vi "FuncVI-APSpectrum.vi"(5 "InstanceRef":T2, 9 "arg list":T1[](array[typedef]) {"num" format="%.2f"}) -> (0 "error out":bool, 3 "result":T1 {"num" format="%.2f"})   [LabVIEW 2021]
doc: "::: CalcExpress Toolkit :::\nCopyright (c) 2000-2026 Konstantin Shifershteyn. All rights reserved."
uses:
  cetypes.llb/CalcExpress Function Argument Info.ctl
  cetypes.llb/CalcExpress Instance RefNum.ctl
  <vilib>/Analysis/NI_AALPro.lvlib
panel:
  in  "max arg num":i32=3
  in  "min arg num":i32=2
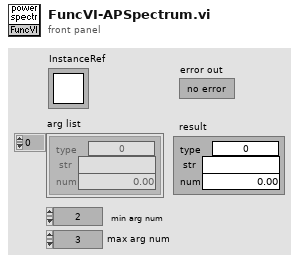
[diagram p1: front panel]
types:
  T1 = typedef "CalcExpress Function Argument Info.ctl" = cluster{"type":u32, "str":string, "num":dbl}
  T2 = typedef "CalcExpress Instance RefNum.ctl" = refnum<k1>
  T3 = enum8{"String", "DBL Number", "identifier", "1D Array of DBL", "2D Array of DBL", "CDB Number", "1D Array of CDB", "2D Array of CDB", "1D Array of String", "2D Array of String", "Unknown data type"}
  T4 = cluster{"index":i32, "type":enum8{"String", "DBL Number", "identifier", "1D Array of DBL", "2D Array of DBL", "CDB Number", "1D Array of CDB", "2D Array of CDB", "Unknown data type"}, "default num":dbl, "default str":string}[]
  T5 = typedef "VarMan Variable Context Handle.ctl" = i32
  T6 = cluster{"type":enum8{"String", "DBL Number", "identifier", "1D Array of DBL", "2D Array of DBL", "CDB Number", "1D Array of CDB", "2D Array of CDB", "1D Array of String", "2D Array of String", "Unknown data type"}, string, "df":dbl}
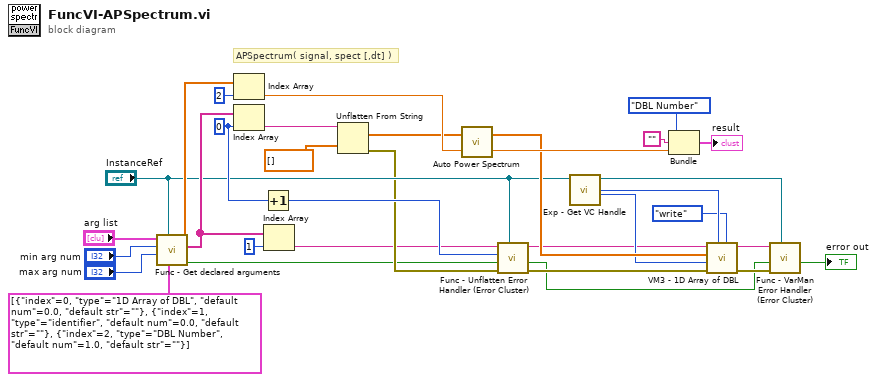
[diagram p0: block diagram]
diagram:
  w19 = 0
  # "APSpectrum( signal, spect [,dt] )"
  n1 = call "Func - Get declared arguments.vi"("arg descriptors"=T4 [{"index"=0, "type"=enum."1D Array of DBL", "default num"=0.0, "default str"=""}, {"index"=1, "type"=enum."identifier", "default num"=0.0, "default str"=""}, {"index"=2, "type"=enum."DBL Number", "default num"=1.0, "default str"=""}] ("args descriptors"), "InstanceRef"="InstanceRef", "max arg num"="max arg num", "min arg num"="min arg num", "arg list"="arg list") -> ("error out"=w5:bool, "str list"=w27:string[], "num list"=w25:dbl[])  [unwired: 3 in, 1 out]
  n2 = Index Array(array=w25, index=2) -> (element=w26:dbl)
  n3 = Index Array(array=w27, index=w19) -> (element=w22:string)
  n4 = Increment(x=w19) -> (x+1=w7:i32)
  n5 = Index Array(array=w27, index=1) -> (element=w4:string)
  n6 = Unflatten From String(type=dbl[] [] ("num list"), binary string=w22) -> (value=w20:dbl[], error out=w6:errorcluster)  [unwired: 3 in, 1 out]
  n7 = call <vilib>:"Auto Power Spectrum.vi"("dt"=w26, "Signal (V)"=w20) -> ("df"=w31:dbl, "Power Spectrum (V^2 rms)"=w14:dbl[])
  n8 = call "Func - Unflatten Error Handler (Error Cluster).vi"("InstanceRef"="InstanceRef", "Unflatten Error Cluster"=w6, "error status before"=w5, "argument number"=w7, "name"=w4) -> ("Error Cluster out"=w9:errorcluster, "error status out"=w1:bool, "dup name"=w3:string)  [unwired: 4 in]
  n9 = call "Exp - Get VC Handle.vi"("InstanceRef"="InstanceRef") -> ("writer ID"=w13:u32, "dup InstanceRef"=w10:T2, "VC Handle"=w16:T5)  [unwired: 5 in, 1 out]
  n10 = Bundle("type"=T3."DBL Number", "", "df"=w31) -> (→"result":T6)  [unwired: 1 in]
  n11 = call "VM3 - 1D Array of DBL.vi"("cmd (read)"=enum16{"create", "destroy", "write", "read"}."write", "VC Handle"=w16, "error in"=w9, "writer ID"=w13, "value in"=w14, "name_spec"=w3) -> ("error out"=w11:errorcluster, "dup name_spec"=w12:string)  [unwired: 2 in, 2 out]
  n12 = call "Func - VarMan Error Handler (Error Cluster).vi"("InstanceRef"=w10, "VarMan VI error in"=w11, "error status before"=w1, "var name"=w12) -> ("FuncVI error out"=→"error out":bool)  [unwired: 5 in, 2 out]
